vi "Refresh Statistics.vi"(11 "CIFPlugin in":refnum<class "CAN_Writer_CANsub_Plugin.lvclass">) -> (3 "CIFPlugin out":refnum<class "CAN_Writer_CANsub_Plugin.lvclass">)   [LabVIEW 2021, in "CAN_Writer_CANsub_Plugin.lvclass"]
uses:
  CAN_Writer_CANsub_Plugin.lvclass
  CAN_Writer_CANsub_Plugin.lvclass/CAN_Writer_CANsub_Plugin.ctl
  Typedef/Statistics.ctl
  <vilib>/CIF Foundation/CIF CAN RW Core/CAN_RW_CORE.lvclass
  <vilib>/CIF Foundation/CIF XNET CAN RW/XNET CAN RW.lvclass
  C:/Program Files/National Instruments/LabVIEW 2021/vi.lib/CIF Foundation/CIF CAN RW Core/CAN_RW_CORE.lvclass
  C:/Program Files/National Instruments/LabVIEW 2021/vi.lib/CIF Foundation/CIF XNET CAN RW/XNET CAN RW.lvclass
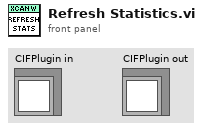
[diagram p1: front panel]
types:
  T1 = typedef "CAN_Writer_CANsub_Plugin.lvclass/Statistics.ctl" = cluster{"Iterations":u64, "FIFO Read Timeouts":u64, "Writen Frames":u64, "Frames Filtered":u64, "FIFO Drops":u64, "ACK Errors":u64}
  T2 = typedef "CAN_RW_CORE.lvclass/Statistics.ctl" = cluster{"Total Frames RW":u32, "Frames Filtered ":u32, "ACK Errors":u32}
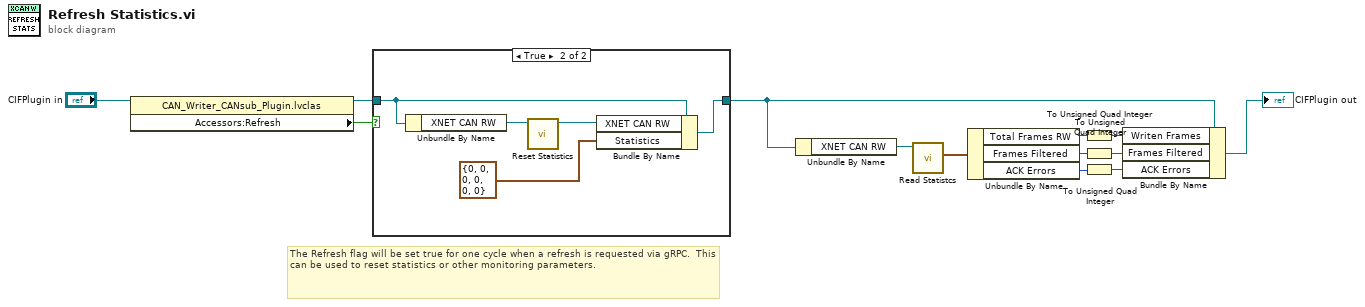
[diagram p0: block diagram]
diagram:
  # "The Refresh flag will be set true for one cycle when a refresh is requested via gRPC.  This can be used to reset statistics or other monitoring parameters."
  n1 = property class="CAN_Writer_CANsub_Plugin.lvclas"(reference="CIFPlugin in") -> (reference out=w11:refnum<class "CAN_Writer_CANsub_Plugin.lvclass">, "Accessors:Refresh"=w12:bool)  [unwired: 1 in, 1 out]
  n2 = case shown="True" w12 {
    tunnel: w11 -> [w14 w17]
    tunnel: [w14 w19] -> w3
    frame False {
    }
    frame True {
      n3 = Unbundle By Name(w17) -> ("XNET CAN RW"=w16:refnum<class "XNET CAN RW.lvclass">)
      n4 = call <vilib>:"Reset Statistics.vi"("CAN_RW_CORE in"=w16) -> ("CAN_RW_CORE out"=w15:refnum<class "XNET CAN RW.lvclass">)  [unwired: 9 in, 1 out]
      n5 = Bundle By Name(cluster=w17, "XNET CAN RW"=w15, "Statistics"=T1 {"Iterations"=0, "FIFO Read Timeouts"=0, "Writen Frames"=0, "Frames Filtered"=0, "FIFO Drops"=0, "ACK Errors"=0} ("-> gRPC Comm.Cyclic Data -> gRPC .Statistics")) -> (w19:refnum<class "CAN_Writer_CANsub_Plugin.lvclass">)
    }
  }
  n6 = Unbundle By Name(w3) -> ("XNET CAN RW"=w5:refnum<class "XNET CAN RW.lvclass">)
  n7 = call <vilib>:"Read Statistcs.vi"("CAN_RW_CORE in"=w5) -> ("Statistcs"=w10:T2)  [unwired: 8 in, 2 out]
  n8 = Unbundle By Name(w10) -> ("Total Frames RW"=w8:u32, "Frames Filtered"=w9:u32, "ACK Errors"=w1:u32)
  n9 = To Unsigned Quad Integer(1:w8) -> (0:w7:u64)
  n10 = To Unsigned Quad Integer(1:w9) -> (0:w6:u64)
  n11 = To Unsigned Quad Integer(1:w1) -> (0:w2:u64)
  n12 = Bundle By Name(cluster=w3, "Writen Frames"=w7, "Frames Filtered"=w6, "ACK Errors"=w2) -> (→"CIFPlugin out":refnum<class "CAN_Writer_CANsub_Plugin.lvclass">)
